vi "_CFX_Sole.vi"(0 "CFX cmd":T7, 1 "CFX State":T1, 5 "CFX-config":T3={"neme"="上板机", "CFX Handle"="Cleaner", "Request IP"="amqp://192.168.1.10:5672", "User"="admin", "password"="123456", "Broker IP"="192.168.1.20", "Broker Port"="5672", "Publish Path"="/exchange/Cleaner", "SubPubish Path"="/queue/Broadcast-Cleaner", "Broadcast \nPublish Path"="/exchange/CFX.Host", "Broadcast Sub\npublish Path"="/queue/Broadcast-CFX.Host", "Target \nHandle lD"="CFX.Host", "target IP"="amqp://127.0.0.1", "unit verification"=TRUE, "heartbeat"=FALSE, "timeout period"=5.0}, 7 "CfxData":T2={"Vendor"="YXD", "UniqueIdentifier"="UID5620001", "FriendlyName"="SBJ", "ModelNumber"="SBJ_0001", "SerialNumber"="563210", "NumberofLanes"="2", "CodeIn"="", "CodeOut"="", "Unitldentifer"="", "PositionNumber"="", "PositionName"="", "OldState"="", "NewState"="", "OldStateDuration"="", "Faultcode"="", "Operatorldentifer"="", "LoginName"="", "RecipeName"="", "Revision"="", "Activate formula"="", "Description"=""}, 11 "Error In":errorcluster caption="错误输入", 12 "send?":bool, 13 "request?":bool) -> (6 "MessageCFX_out":string, 8 "CFX_Message_In":T4, 14 "ok?":bool, 15 "Error Out":errorcluster caption="错误输出")   [LabVIEW 2025]
uses:
  CFX_dll/CFX.dll
  ctl/CFX-cmd.ctl
  ctl/CfxTopic-cmd.ctl
  ctl/CFX_data.ctl
  ctl/CFX-config.ctl
  SubVI/table/1 model/a log/_myType runlog cmd.ctl
panel:
  out "cmd State":T1=enum."Event"
  in  "Sole?":bool
  out "QueueName":string
  out "IsOpen":bool
  in  "CFX.Host?":bool
  in  "enable?":bool
  out "TraceMessage_EVE":refnum<k27>
  out "TraceMessage":string
  out "AooLog":refnum<k24>
  out "TestSubscribeChannel":bool
  out "TestPublishChannel":bool
  out "log":string
  out "error out":errorcluster
  out "objAMQP_MSG":refnum<k27>
  out "Connection":T5 {"ConnectionEstablished" items=["ConnectionEstablished", "ConnectionFailed", "ConnectionInterrupted", "ConnectionClosed"]}
  out "objAMQP_Request":refnum<k27>
  out "SubscribeChannel":refnum<k24>
  out "return":T6={"CFXHandle"="Cleaner", "RequestNetworkUri"="amqp://10.33.191.97:5672", "RequestTargetAddress"="/queue/Cleaner", "CFX_Message_In"={"Message_Name"="", "Message_Content"=""}, "CFX_Message_out"={"Message_Name"="", "Message_Content"=""}, "CFX_data"=refnum}
  out "FromListener":string
  in  "EndpointInformation":string
  in  "NewState":i32(ring)=1000 items=["PRD"=1000, "PRD_RegularWork"=1100, "PRD_WorkForThirdParties"=1200, "PRD_Rework"=1300, "PRD_Engineering"=1400, "SBY"=2000, "SBY_NoOperator"=2100, "SBY_NoProduct"=2200, "SBY_NoSupportTool"=2300, "SBY_AssociatedClusterModuleDown"=2400, "SBY_NoHost"=2500, "ENG"=3000, "ENG_ProcessExperiments"=3100, "ENG_EquipmentExperiments"=3200, "SDT"=4000, "SDT_UserMaintenanceDelay"=4100, "SDT_SuppliedMaintenanceDelay"=4200, "SDT_PreventiveMaintenance"=4300, "SDT_ChangeOfConsumables"=4400, "SDT_Setup"=4500, "SDT_ProductionTest"=4600, "SDT_FacilitiesRelated"=4700, "USD"=5000, "USD_UserMaintentanceDelay"=5100, "USD_SuppliedMaintenanceDelay"=5200, "USD_Repair"=5300, "USD_OutOfSpecInputMaterial"=5400, "USD_ChangeOfConsumables"=5500, "USD_FacilitiesRelated"=5600, "NST"=6000, "NST_UnworkedShifts"=6100, "NST_EquipmentInstallation"=6200, "NST_EquipmentModifications"=6300, "NST_OfflineTraining"=6400, "NST_ShutdownAndStartup"=6500]
  in  "Broker Url":string="amqp://admin:123456@10.33.191.54:5672"
  out "PublishChannel":refnum<k24>
  in  "rngNewState":i32(ring) items=["PRD"=1000, "PRD_RegularWork"=1100, "PRD_WorkForThirdParties"=1200, "PRD_Rework"=1300, "PRD_Engineering"=1400, "SBY"=2000, "SBY_NoOperator"=2100, "SBY_NoProduct"=2200, "SBY_NoSupportTool"=2300, "SBY_AssociatedClusterModuleDown"=2400, "SBY_NoHost"=2500, "ENG"=3000, "ENG_ProcessExperiments"=3100, "ENG_EquipmentExperiments"=3200, "SDT"=4000, "SDT_UserMaintenanceDelay"=4100, "SDT_SuppliedMaintenanceDelay"=4200, "SDT_PreventiveMaintenance"=4300, "SDT_ChangeOfConsumables"=4400, "SDT_Setup"=4500, "SDT_ProductionTest"=4600, "SDT_FacilitiesRelated"=4700, "USD"=5000, "USD_UserMaintentanceDelay"=5100, "USD_SuppliedMaintenanceDelay"=5200, "USD_Repair"=5300, "USD_OutOfSpecInputMaterial"=5400, "USD_ChangeOfConsumables"=5500, "USD_FacilitiesRelated"=5600, "NST"=6000, "NST_UnworkedShifts"=6100, "NST_EquipmentInstallation"=6200, "NST_EquipmentModifications"=6300, "NST_OfflineTraining"=6400, "NST_ShutdownAndStartup"=6500]
  # "此端点的唯一 CFX 句柄。"
  # "节点队列名"
  # "amqp://10.33.191.64:5672"
  # "Laser"
  # "amqp://localhost:5672"
  # "amqp://192.168.1.20:5672"
  # "Local Request Uri"
  # "amqp://10.33.191.64:5688"
  # "AMQP 源或目标的网络地址。可以包括 user 和 port 信息 标准 Uri 格式。（例如：amqps://user1:password1@myamqpbroker.company1.com、amqp://broker3.company1.com、 amqps://myamqpbroker.company1.com:8856 等）。"
  # "本地消息源\nRequest Source"
  # "代理层\nBroker"
  # "请求目标\nRequest Target"
  # "可配置项"
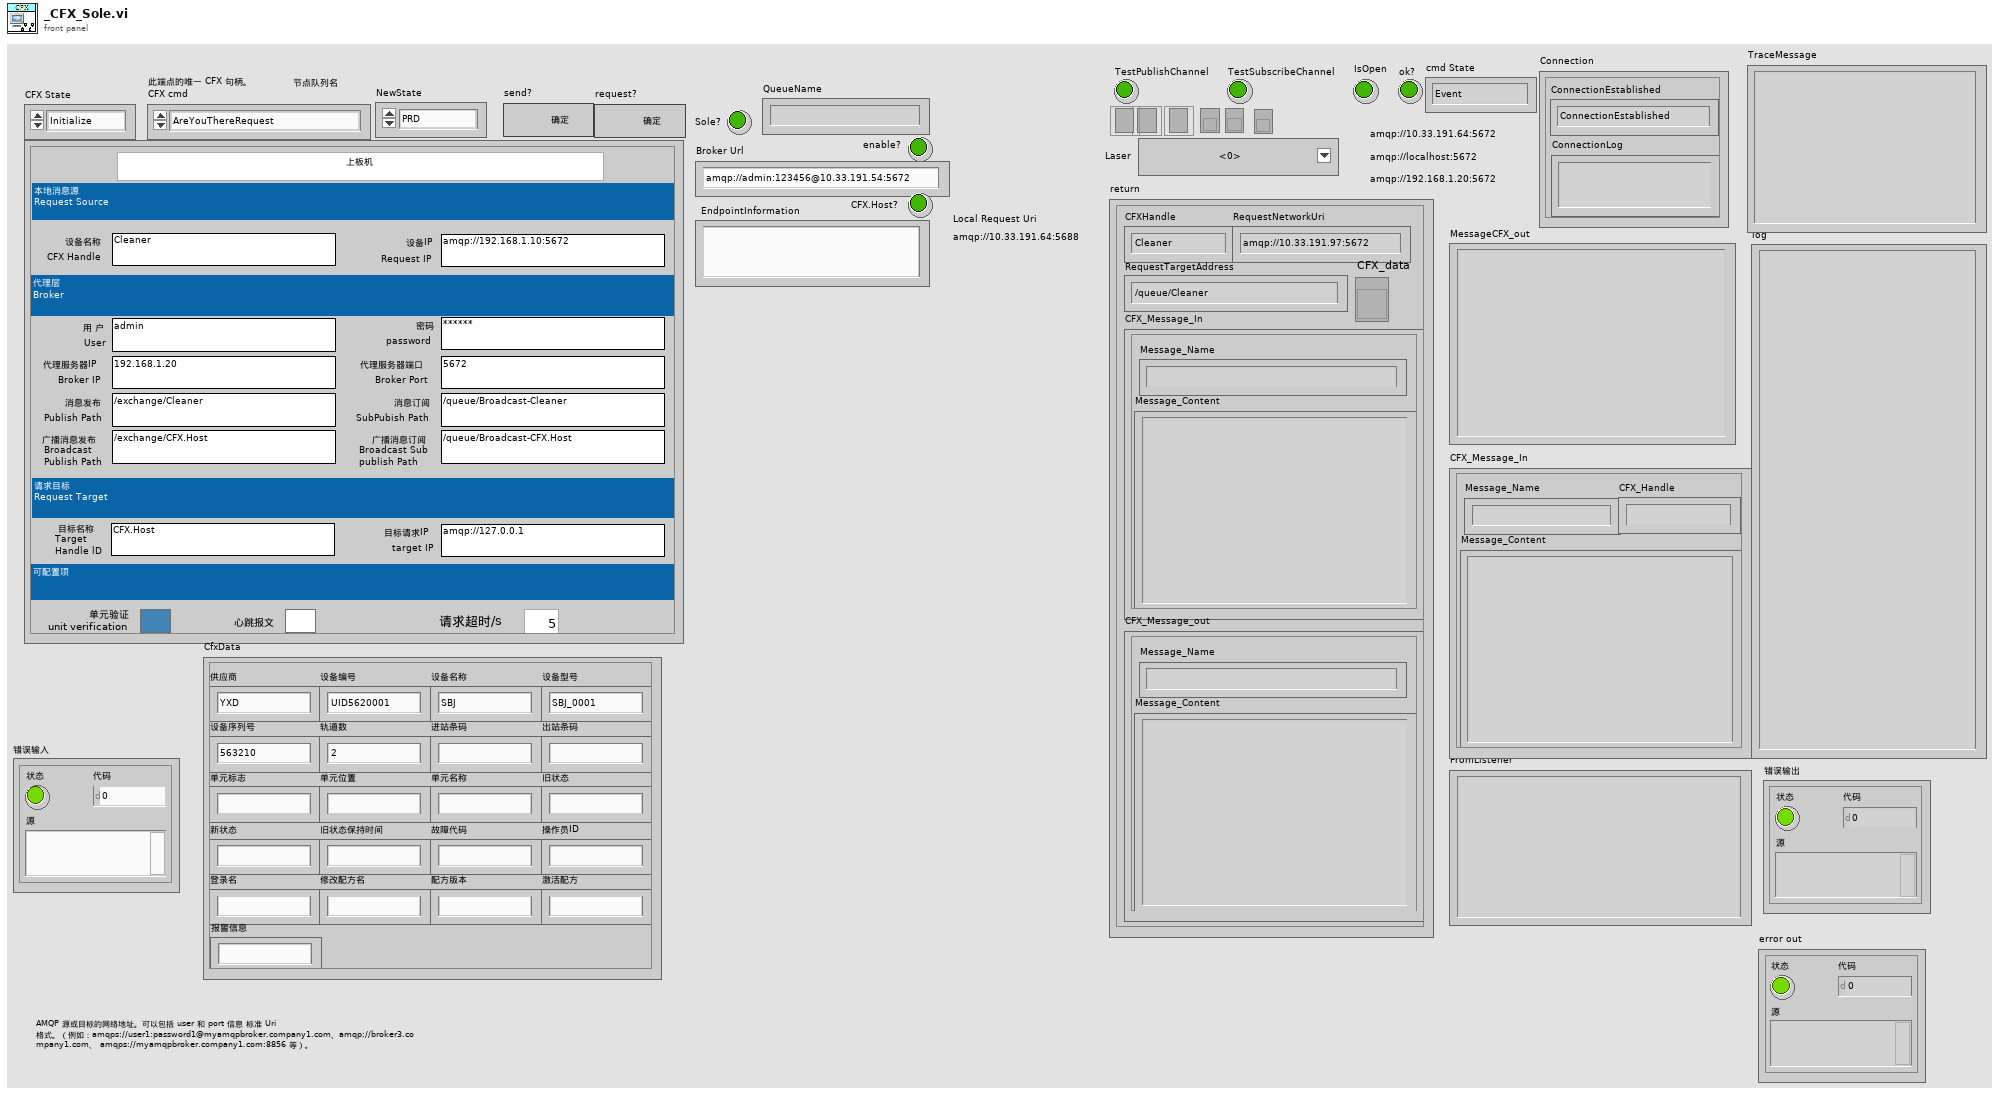
[diagram p1: front panel]
types:
  T1 = typedef "CFX-cmd.ctl" = enum16{"Initialize", "Event", "Connection test", "OpenConnection", "Idle", "Shutdown", "WorkComplete", "StationStateChanged", "MaterialsApplied", "CFX", "Hermes"}
  T2 = typedef "CFX_data.ctl" = cluster{"Vendor":string, "UniqueIdentifier":string, "FriendlyName":string, "ModelNumber":string, "SerialNumber":string, "NumberofLanes":string, "CodeIn":string, "CodeOut":string, "Unitldentifer":string, "PositionNumber":string, "PositionName":string, "OldState":string, "NewState":string, "OldStateDuration":string, "Faultcode":string, "Operatorldentifer":string, "LoginName":string, "RecipeName":string, "Revision":string, "Activate formula":string, "Description":string}
  T3 = typedef "CFX-config.ctl" = cluster{"neme":string, "CFX Handle":string, "Request IP":string, "User":string, "password":string, "Broker IP":string, "Broker Port":string, "Publish Path":string, "SubPubish Path":string, "Broadcast \nPublish Path":string, "Broadcast Sub\npublish Path":string, "Target \nHandle lD":string, "target IP":string, "unit verification":bool, "heartbeat":bool, "timeout period":dbl}
  T4 = cluster{"Message_Name":string, "CFX_Handle":string, "Message_Content":string}
  T5 = cluster{"ConnectionEstablished":i32, "ConnectionLog":string}
  T6 = cluster{"CFXHandle":string, "RequestNetworkUri":string, "RequestTargetAddress":string, "CFX_Message_In":cluster{"Message_Name":string, "Message_Content":string}, "CFX_Message_out":cluster{"Message_Name":string, "Message_Content":string}, "CFX_data":refnum<vi>}
  T7 = typedef "CfxTopic-cmd.ctl" = enum16{"AreYouThereRequest", "AreYouThereResponse", "EndpointConnected", "EndpointShuttingDown", "GetEndpointInformationRequest", "GetEndpointInformationResponse", "Heartbeat", "NotSupportedResponse", "WhoIsThereRequest", "WhoIsThereResponse", "UnitArrived", "UnitsDeparted", "StationStateChanged", "FaultOccurred", "FaultCleared", "OperatorActivated", "OperatorDeactivated", "RecipeModified", "RecipeActived", "ActivateRecipeRequest", "ActivateRecipeResponse"}
  T8 = typedef "_myType runlog cmd.ctl" = enum16{"init", "push (-1: error)", "push (0: user)", "push (1: logical)", "push (2: driver)", "push (3: lib-core)", "push (4: reserved)", "pop", "more?"}
  T9 = typedef "LVStringsAndValuesArrayTypeDef_I32.ctl" = cluster{"String":string, "Value":i32}[]
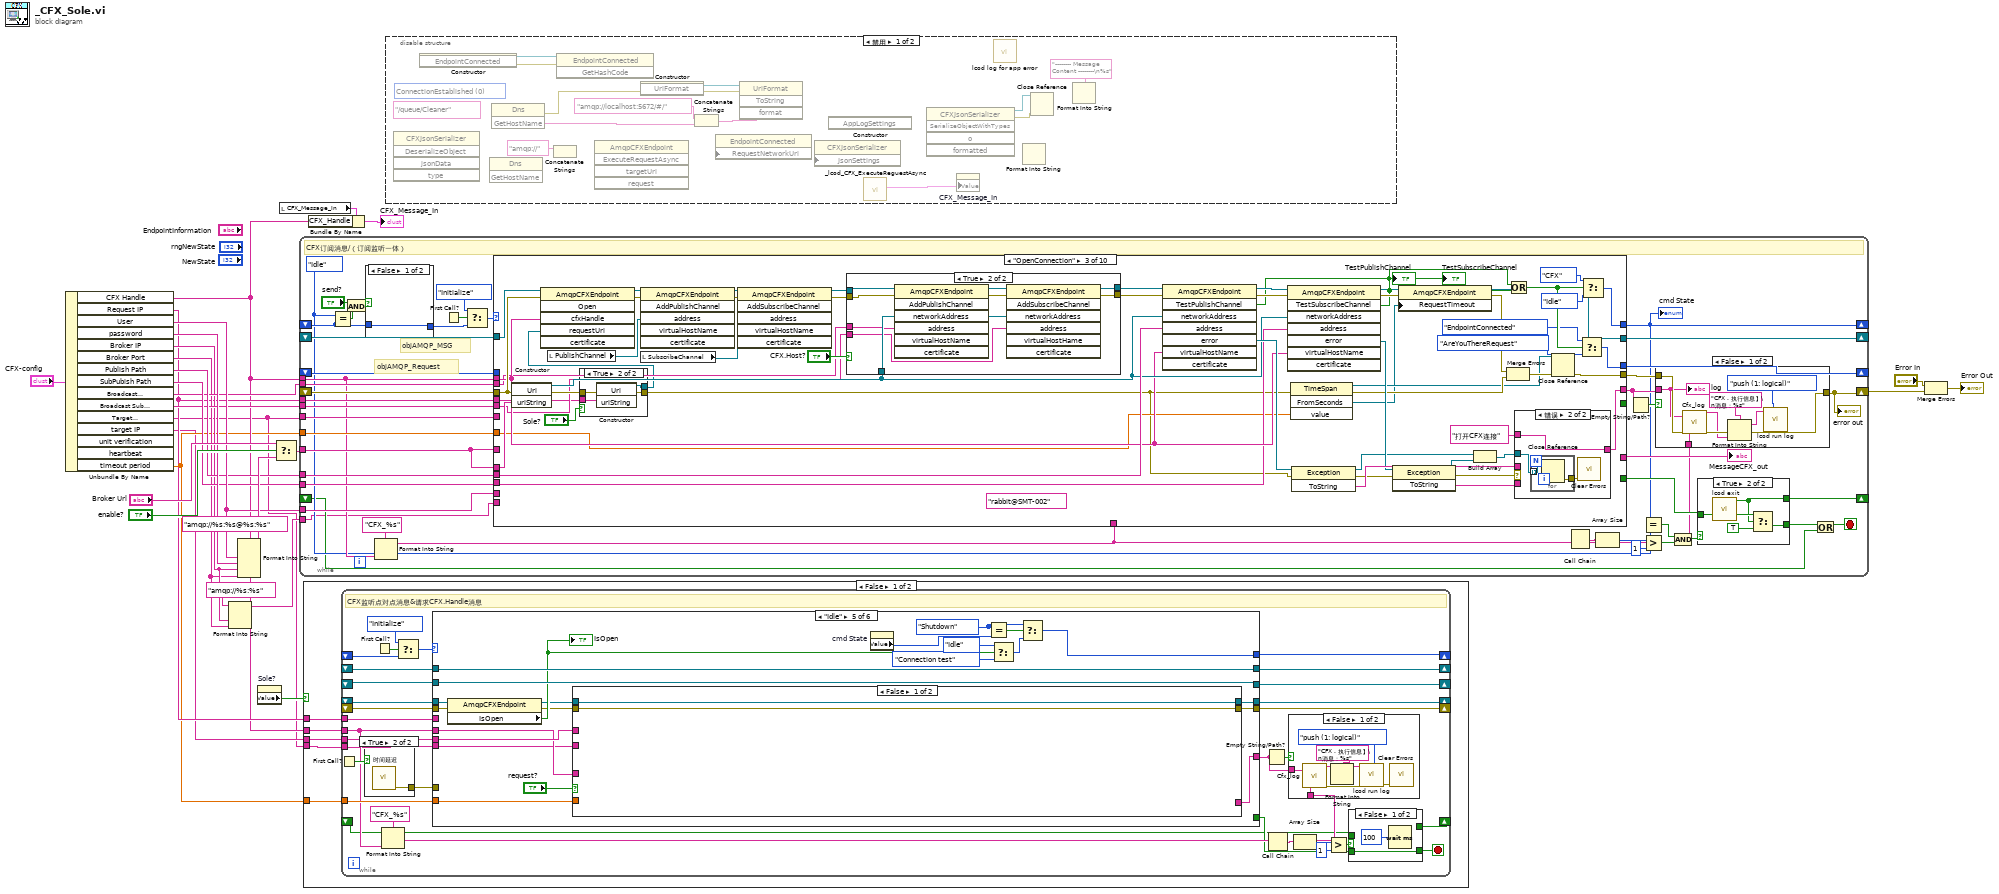
[diagram p0: block diagram]
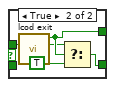
[diagram p2: hidden frame]
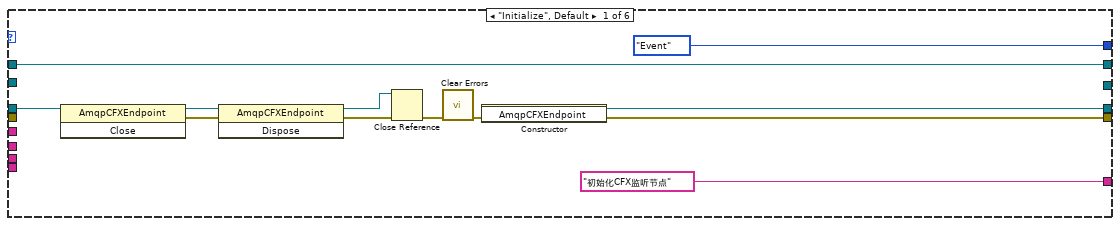
[diagram p5: hidden frame]
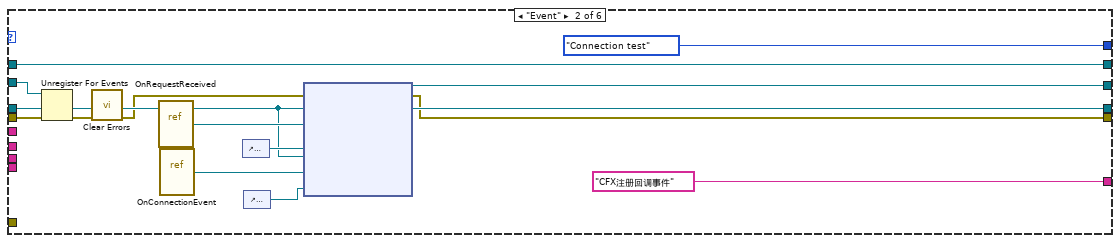
[diagram p6: hidden frame]
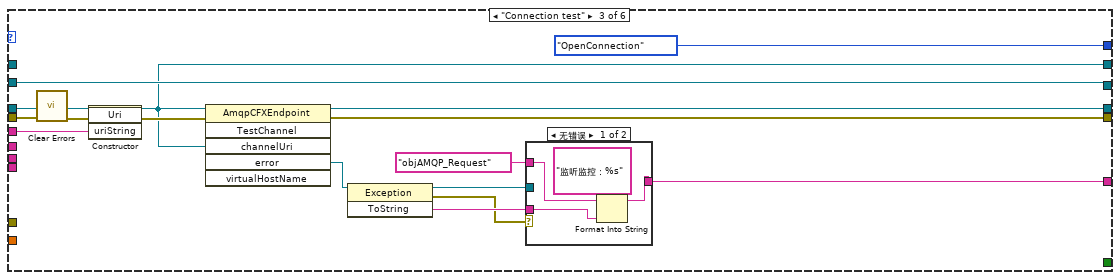
[diagram p7: hidden frame]
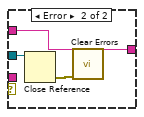
[diagram p8: hidden frame]
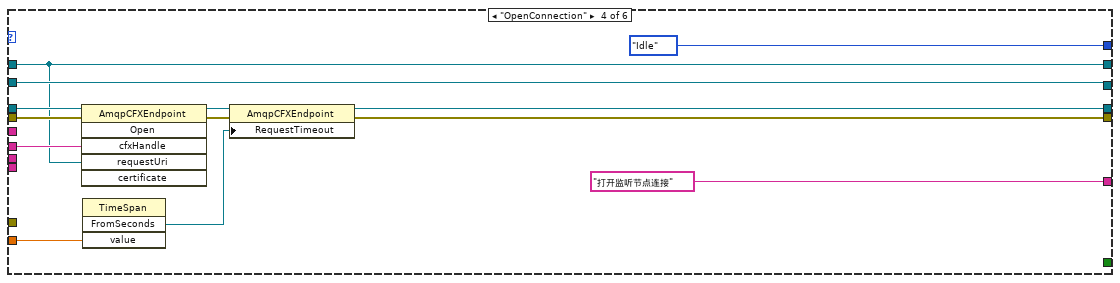
[diagram p9: hidden frame]
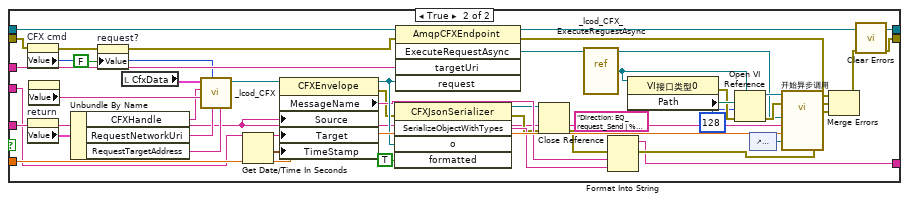
[diagram p10: hidden frame]
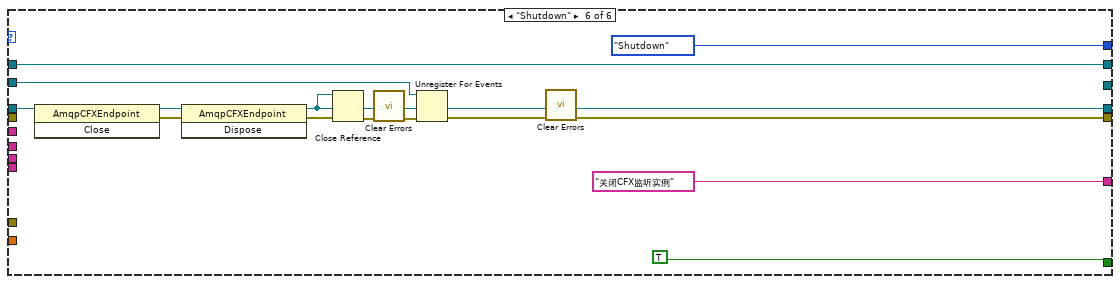
[diagram p11: hidden frame]
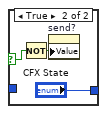
[diagram p14: hidden frame]
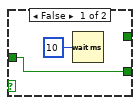
[diagram p15: hidden frame]
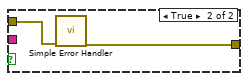
[diagram p16: hidden frame]
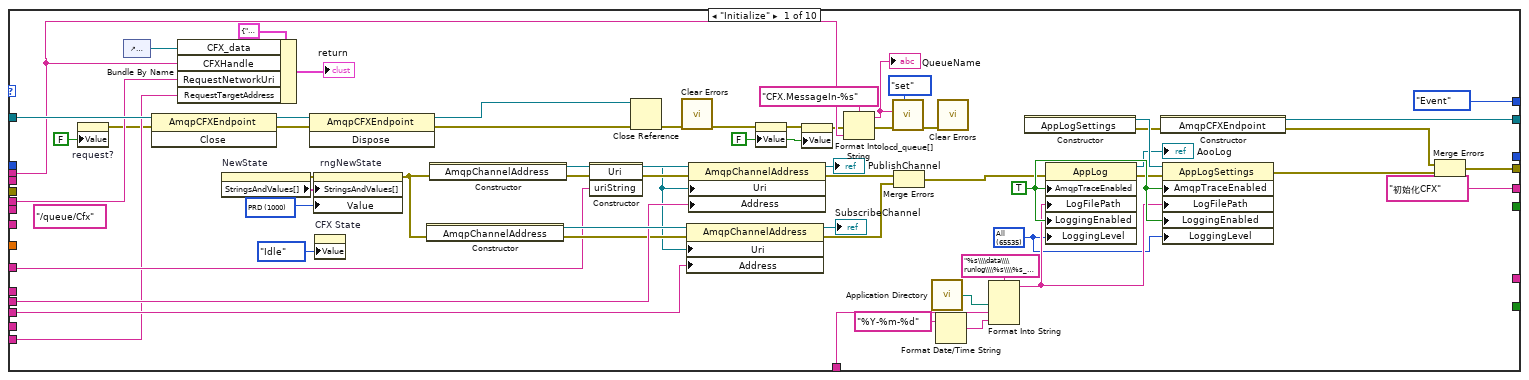
[diagram p17: hidden frame]
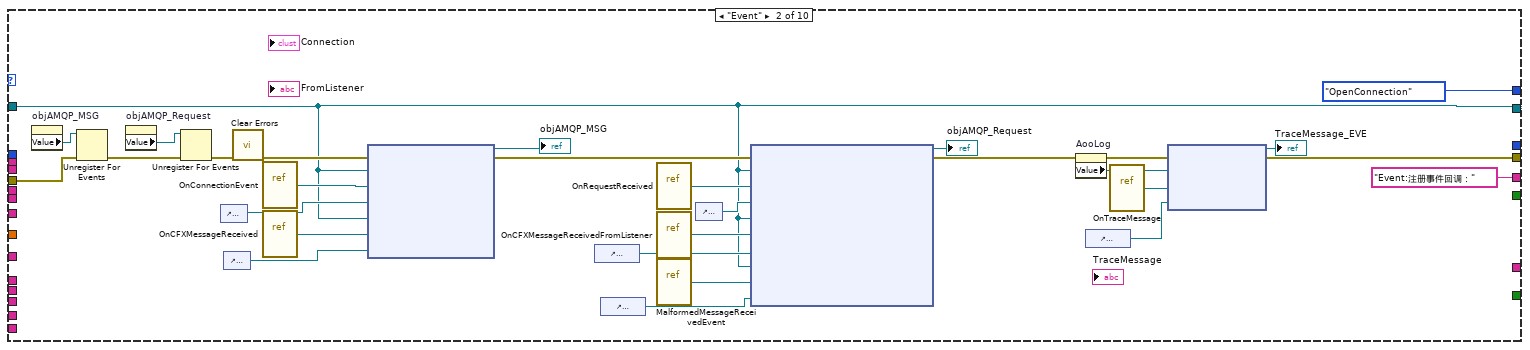
[diagram p18: hidden frame]
diagram:
  n1 = Unbundle By Name("CFX-config") -> ("CFX Handle"=w5:string, "Request IP"=w6:string, "User"=w20:string, "password"=w19:string, "Broker IP"=w10:string, "Broker Port"=w9:string, "Publish Path"=w18:string, "SubPubish Path"=w17:string, "Broadcast \nPublish Path"=w16:string, "Broadcast Sub\npublish Path"=w15:string, "Target \nHandle lD"=w1:string, "target IP"=w2:string, "timeout period"=w4:dbl)  [unwired: 2 out]
  n2 = Format Into String(format string="amqp://%s:%s" ("格式字符串"), w10, w9) -> (resulting string=w8:string)  [unwired: 2 in, 1 out]
  n3 = Format Into String(format string="amqp://%s:%s@%s:%s" ("格式字符串"), w20, w19, w10, w9) -> (resulting string=w22:string)  [unwired: 2 in, 1 out]
  n4 = property on="Sole?" class="Bool (严格)"() -> ("Value"=w3:bool)  [unwired: 2 in, 2 out]
  n5 = Select(t="Broker Url", s="enable?", f=w22) -> (s? t:f=w14:string)
  n6 = local read "CFX_Message_In"() -> (w13:T4)
  n7 = while {
    shift-right: [w47] -> _
    shift-left: _ -> [w36]
    shift-right: [w70] -> _
    shift-left: _ -> [w71]
    shift-right: [w64] -> w7
    shift-left: _ -> [w58]
    shift-right: [w63] -> _
    shift-left: _ -> [w65]
    tunnel: w14 -> [w59]
    tunnel: w17 -> [w62]
    tunnel: w18 -> [w61]
    tunnel: w5 -> [w41]
    tunnel: w20 -> [w60]
    tunnel: w6 -> [w57]
    tunnel: w16 -> [w56]
    tunnel: w15 -> [w55]
    tunnel: w1 -> [w54]
    tunnel: w4 -> [w53]
    shift-right: [w37] -> _
    shift-left: _ -> [w31]
    tunnel: w8 -> [w28]
    stop <- w32 stop-if-true
    w35 = CFX-cmd."Idle" ("CFX State")
    # "objAMQP_Request"
    # "objAMQP_MSG"
    # "CFX订阅消息/（订阅监听一体）"
    n8 = Equal?(x=w35, y=w36) -> (x = y?=w33:bool)
    n9 = And(x="send?", y=w33) -> (x .and. y?=w34:bool)
    n10 = case shown="False" w34 {
      selector: w34 -> [_ w74]
      tunnel: w36 -> [w72 _]
      tunnel: [w72 "CFX State"] -> w40
      frame False {
      }
      frame True {
        n11 = Not(x=w74) -> (.not. x?=w73:bool)
        n12 = property on="send?" class="Bool (严格)"("Value"=w73) -> ()  [unwired: 2 in, 2 out]
      }
    }
    n13 = Format Into String(format string="CFX_%s" ("log_path"), w41) -> (resulting string=w39:string)  [unwired: 2 in, 1 out]
    n14 = First Call?() -> (First Call?: T/F=w29:bool)
    n15 = Select(t=CFX-cmd."Initialize" ("CFX State"), s=w29, f=w40) -> (s? t:f=w43:T1)
    n16 = case shown="\"OpenConnection\"" w43 {
      selector: w43 -> [_ _ _ w294 _ _ _ _ _ _]
      tunnel: [_ _ _ _ w340 _ _ _ _ _] -> w49
      tunnel: w71 -> [w132 w153 w237 w283 w346 w390 w418 w443 w483 w501]
      tunnel: [w138 w153 w194 w269 w342 w389 w416 w442 w482 w500] -> w70
      tunnel: [w133 w172 w208 errorcluster {"status"=FALSE, "code"=0, "source"=""} ("error out") w341 w386 w413 w441 w493 w499] -> w69
      tunnel: [_ _ _ w293 _ w381 w405 w428 w477 w498] -> w68
      tunnel: [_ _ _ TRUE _ _ _ _ _ _] -> _
      tunnel: ["初始化CFX" ("格式字符串") "Event:注册事件回调：" ("SerializeObjectWithTypes") w230 "" ("SerializeObjectWithTypes") w345 w378 w405 w427 w487 w498] -> w67
      tunnel: [CFX-cmd."Event" ("CFX State") CFX-cmd."OpenConnection" ("CFX State") w201 w278 w344 CFX-cmd."Idle" ("CFX State") CFX-cmd."Idle" ("CFX State") CFX-cmd."Idle" ("CFX State") w463 CFX-cmd."Idle" ("CFX State")] -> w47
      tunnel: w58 -> [_ w167 w211 w266 w343 w376 w403 w425 w484 w496]
      tunnel: w65 -> [_ _ _ _ w339 _ _ _ w467 _]
      tunnel: [_ _ w197 w288 w336 _ _ _ w462 _] -> w63
      tunnel: w59 -> [w105 _ _ _ _ _ _ _ _ _]
      tunnel: w62 -> [w123 _ w190 _ _ _ _ _ _ _]
      tunnel: w61 -> [w122 _ w220 w285 _ _ _ _ _ _]
      tunnel: w41 -> [w108 _ w204 _ _ _ _ _ w460 _]
      tunnel: w60 -> [_ _ _ w284 _ _ _ _ _ _]
      tunnel: w59 -> [_ _ w219 _ _ _ _ _ _ _]
      tunnel: w57 -> [w109 _ w188 _ _ _ _ _ _ _]
      tunnel: w56 -> [_ _ w192 _ _ _ _ _ _ _]
      tunnel: w55 -> [_ _ w191 _ _ _ _ _ _ _]
      tunnel: w54 -> [_ _ _ _ _ _ _ _ w459 _]
      tunnel: w53 -> [_ _ w189 _ _ _ _ _ _ _]
      tunnel: w39 -> [w107 _ _ _ _ _ _ _ _ _]
      tunnel: w28 -> [w98 _ _ _ _ _ _ _ _ _]
      frame "Initialize" {
        (unwired) "/queue/Cfx" ("RequestTargetAddress")
        w127 = FALSE ("TestPublishChannel")
        w135 = 65535 items=["Debug"=1, "Info"=2, "Warn"=4, "Error"=8, "All"=65535] ("LoggingLevel")
        w137 = TRUE ("LoggingEnabled")
        w149 = 1000 items=["PRD"=1000, "PRD_RegularWork"=1100, "PRD_WorkForThirdParties"=1200, "PRD_Rework"=1300, "PRD_Engineering"=1400, "SBY"=2000, "SBY_NoOperator"=2100, "SBY_NoProduct"=2200, "SBY_NoSupportTool"=2300, "SBY_AssociatedClusterModuleDown"=2400, "SBY_NoHost"=2500, "ENG"=3000, "ENG_ProcessExperiments"=3100, "ENG_EquipmentExperiments"=3200, "SDT"=4000, "SDT_UserMaintenanceDelay"=4100, "SDT_SuppliedMaintenanceDelay"=4200, "SDT_PreventiveMaintenance"=4300, "SDT_ChangeOfConsumables"=4400, "SDT_Setup"=4500, "SDT_ProductionTest"=4600, "SDT_FacilitiesRelated"=4700, "USD"=5000, "USD_UserMaintentanceDelay"=5100, "USD_SuppliedMaintenanceDelay"=5200, "USD_Repair"=5300, "USD_OutOfSpecInputMaterial"=5400, "USD_ChangeOfConsumables"=5500, "USD_FacilitiesRelated"=5600, "NST"=6000, "NST_UnworkedShifts"=6100, "NST_EquipmentInstallation"=6200, "NST_EquipmentModifications"=6300, "NST_OfflineTraining"=6400, "NST_ShutdownAndStartup"=6500] ("NewState")
        n17 = property on="request?" class="Bool (严格)"("Value"=FALSE ("request?")) -> (error out=w93:errorcluster)  [unwired: 2 in, 1 out]
        n18 = control-ref of="CfxData"() -> (w95:refnum<vi>)
        n19 = invoke class="AmqpCFXEndpoint" method="Close"(reference=w132, error in=w93) -> (reference out=w130:refnum<k24>, error out=w99:errorcluster)  [unwired: 1 in, 1 out]
        n20 = Bundle By Name(cluster=T6 {"CFXHandle"="Cleaner", "RequestNetworkUri"="amqp://192.168.1.10:5672", "RequestTargetAddress"="/queue/Cleaner", "CFX_Message_In"={"Message_Name"="", "Message_Content"=""}, "CFX_Message_out"={"Message_Name"="", "Message_Content"=""}, "CFX_data"=refnum} ("return"), "CFX_data"=w95, "CFXHandle"=w108, "RequestNetworkUri"=w109, "RequestTargetAddress"=w98) -> (→"return":T6)
        n21 = property on="NewState" class="Ring (严格)"() -> (error out=w148:errorcluster, "StringsAndValues[]"=w152:T9)  [unwired: 2 in, 1 out]
        n22 = invoke on="调用节点" class="AmqpCFXEndpoint" method="Dispose"(reference=w130, error in=w99) -> (reference out=w101:refnum<k24>, error out=w100:errorcluster)  [unwired: 1 in, 1 out]
        n23 = property on="rngNewState" class="Ring (严格)"(error in=w148, "StringsAndValues[]"=w152, "Value"=w149) -> (error out=w129:errorcluster)  [unwired: 1 in, 1 out]
        n24 = property on="CFX State" class="Enum (严格)"("Value"=CFX-cmd."Idle" ("CFX State")) -> ()  [unwired: 2 in, 2 out]
        n25 = constructor class="AmqpChannelAddress"(error in=w129) -> (reference out=w142:refnum<k24>, error out=w121:errorcluster)  [unwired: 2 in, 1 out]
        n26 = constructor class="AmqpChannelAddress"(error in=w129) -> (reference out=w147:refnum<k24>, error out=w151:errorcluster)  [unwired: 2 in, 1 out]
        n27 = constructor class="Uri"(error in=w151, "uriString"=w105) -> (reference out=w120:refnum<k24>, error out=w150:errorcluster)  [unwired: 2 in, 2 out]
        n28 = Close Reference(reference=w101, error in (no error)=w100) -> (error out=w131:errorcluster)
        n29 = call <vilib>:"Clear Errors.vi"("error in (no error)"=w131) -> ("error out"=w119:errorcluster)  [unwired: 5 in, 1 out]
        n30 = property class="AmqpChannelAddress"(reference=w142, error in=w121, "Uri"=w120, "Address"=w123) -> (reference out=→"SubscribeChannel":refnum<k24>, error out=w140:errorcluster)
        n31 = property class="AmqpChannelAddress"(reference=w147, error in=w150, "Uri"=w120, "Address"=w122) -> (reference out=→"PublishChannel":refnum<k24>, error out=w141:errorcluster)
        n32 = property on="TestPublishChannel" class="Bool (严格)"(error in=w119, "Value"=w127) -> (error out=w128:errorcluster)  [unwired: 1 in, 1 out]
        n33 = property on="TestSubscribeChannel" class="Bool (严格)"(error in=w128, "Value"=w127) -> (error out=w104:errorcluster)  [unwired: 1 in, 1 out]
        n34 = Format Into String(format string="CFX.MessageIn-%s" ("格式字符串"), error in=w104, w108) -> (resulting string=w113:string, error out=w110:errorcluster)  [unwired: 1 in]
        "QueueName" <- w113
        n35 = call "locd_queue[].vi"("cmd"=enum16{"init", "get", "set", "end"}."set", "error in"=w110, "queue_name"=w113) -> ("error out"=w111:errorcluster)  [unwired: 4 in, 4 out]
        n36 = Merge Errors(w141, w140) -> (w112:errorcluster)
        n37 = call <vilib>:"Application Directory.vi"() -> ("Application Directory"=w146:path)
        n38 = Format Date/Time String(time format string (%c)="%Y-%m-%d" ("格式字符串")) -> (date/time string=w106:string)  [unwired: 2 in]
        n39 = call <vilib>:"Clear Errors.vi"("error in (no error)"=w111) -> ()  [unwired: 5 in, 2 out]
        n40 = Format Into String(format string="%s\\\\data\\\\runlog\\\\%s\\\\%s_cfxDebig.txt" ("格式字符串"), w146, w107, w106) -> (resulting string=w136:string)  [unwired: 2 in, 1 out]
        n41 = constructor class="AppLogSettings"() -> (reference out=w134:refnum<k24>, error out=w126:errorcluster)  [unwired: 3 in, 1 out]
        n42 = property class="AppLog"(error in=w112, "AmqpTraceEnabled"=w137, "LogFilePath"=w136, "LoggingEnabled"=w137, "LoggingLevel"=w135) -> (reference out=→"AooLog":refnum<k24>, error out=w124:errorcluster)  [unwired: 1 in]
        n43 = constructor class="AmqpCFXEndpoint"(error in=w126) -> (reference out=w138:refnum<k24>, error out=w102:errorcluster)  [unwired: 2 in, 1 out]
        n44 = property class="AppLogSettings"(reference=w134, error in=w124, "AmqpTraceEnabled"=w137, "LogFilePath"=w136, "LoggingEnabled"=w137, "LoggingLevel"=w135) -> (error out=w116:errorcluster)  [unwired: 1 out]
        n45 = Merge Errors(w102, w116) -> (w133:errorcluster)
      }
      frame "Event" {
        n46 = property on="objAMQP_MSG" class="Ref (严格)"() -> ("Value"=w156:refnum<k27>)  [unwired: 2 in, 2 out]
        n47 = Unregister For Events(event registration refnum=w156, error in=w167) -> (error out=w157:errorcluster)
        n48 = property on="objAMQP_Request" class="Ref (严格)"() -> ("Value"=w154:refnum<k27>)  [unwired: 2 in, 2 out]
        n49 = Unregister For Events(event registration refnum=w154, error in=w157) -> (error out=w155:errorcluster)
        n50 = control-ref of="Connection"() -> (w179:refnum<vi>)
        n51 = control-ref of="CFX_Message_In"() -> (w164:refnum<vi>)
        n52 = call <vilib>:"Clear Errors.vi"("error in (no error)"=w155) -> ("error out"=w158:errorcluster)  [unwired: 5 in, 1 out]
        n53 = vi-ref "OnConnectionEvent.vi"() -> ("vi reference"=w180:refnum<vi>)
        n54 = vi-ref "OnCFXMessageReceived.vi"() -> ("vi reference"=w165:refnum<vi>)
        n55 = node(w158, w153, w180, w179, w153, w165, w164) -> (→"objAMQP_MSG":refnum<k27>, w163:errorcluster)  [unwired: 1 in]
        n56 = control-ref of="FromListener"() -> (w161:refnum<vi>)
        n57 = control-ref of="FromListener"() -> (w159:refnum<vi>)
        n58 = vi-ref "OnRequestReceived.vi"() -> ("vi reference"=w178:refnum<vi>)
        n59 = vi-ref "OnCFXMessageReceivedFromListener.vi"() -> ("vi reference"=w162:refnum<vi>)
        n60 = vi-ref "MalformedMessageReceivedEvent.vi"() -> ("vi reference"=w160:refnum<vi>)
        n61 = control-ref of="return"() -> (w169:refnum<vi>)
        n62 = node(w163, w153, w178, w169, w153, w162, w161, w153, w160, w159) -> (→"objAMQP_Request":refnum<k27>, w166:errorcluster)  [unwired: 1 in]
        n63 = property on="AooLog" class="Ref (严格)"(error in=w166) -> (error out=w168:errorcluster, "Value"=w174:refnum<k24>)  [unwired: 1 in, 1 out]
        n64 = control-ref of="TraceMessage"() -> (w170:refnum<vi>)
        n65 = vi-ref "OnTraceMessage.vi"() -> ("vi reference"=w173:refnum<vi>)
        n66 = node(w168, w174, w173, w170) -> (→"TraceMessage_EVE":refnum<k27>, w172:errorcluster)  [unwired: 1 in]
      }
      frame "OpenConnection" {
        (unwired) "rabbit@SMT-002" ("sourceAddress")
        n67 = constructor class="Uri"(error in=w211, "uriString"=w219) -> (reference out=w218:refnum<k24>, error out=w216:errorcluster)  [unwired: 2 in, 2 out]
        n68 = local read "PublishChannel"() -> (w232:refnum<k24>)
        n69 = case shown="True" "Sole?" {
          tunnel: w216 -> [w238 w242]
          tunnel: w188 -> [_ w241]
          tunnel: [_ w240] -> w184
          tunnel: [w238 w239] -> w183
          frame False {
          }
          frame True {
            n70 = constructor class="Uri"(error in=w242, "uriString"=w241) -> (reference out=w240:refnum<k24>, error out=w239:errorcluster)  [unwired: 2 in, 2 out]
          }
        }
        n71 = invoke class="AmqpCFXEndpoint" method="Open"(reference=w237, error in=w211, "cfxHandle"=w204, "requestUri"=w184) -> (reference out=w215:refnum<k24>, error out=w214:errorcluster)  [unwired: 2 in, 4 out]
        n72 = local read "SubscribeChannel"() -> (w233:refnum<k24>)
        n73 = invoke class="AmqpCFXEndpoint" method="AddPublishChannel"(reference=w215, error in=w214, "address"=w232) -> (reference out=w236:refnum<k24>, error out=w235:errorcluster)  [unwired: 3 in, 4 out]
        n74 = invoke class="AmqpCFXEndpoint" method="AddSubscribeChannel"(reference=w236, error in=w235, "address"=w233) -> (reference out=w212:refnum<k24>, error out=w205:errorcluster)  [unwired: 3 in, 4 out]
        n75 = case shown="True" "CFX.Host?" {
          tunnel: w218 -> [_ w253]
          tunnel: [w243 w252] -> w217
          tunnel: [w244 w251] -> w213
          tunnel: w212 -> [w244 w250]
          tunnel: w205 -> [w243 w247]
          tunnel: w192 -> [_ w246]
          tunnel: w191 -> [_ w245]
          frame False {
          }
          frame True {
            n76 = invoke class="AmqpCFXEndpoint" method="AddPublishChannel"(reference=w250, error in=w247, "networkAddress"=w253, "address"=w246) -> (reference out=w248:refnum<k24>, error out=w249:errorcluster)  [unwired: 3 in, 5 out]
            n77 = invoke class="AmqpCFXEndpoint" method="AddSubscribeChannel"(reference=w248, error in=w249, "networkAddress"=w253, "address"=w245) -> (reference out=w251:refnum<k24>, error out=w252:errorcluster)  [unwired: 3 in, 5 out]
          }
        }
        n78 = invoke on="调用节点" class="AmqpCFXEndpoint" method="TestPublishChannel"(reference=w213, error in=w217, "networkAddress"=w218, "address"=w220, "virtualHostName"=w204) -> (reference out=w231:refnum<k24>, error out=w222:errorcluster, "TestPublishChannel"=w203:bool, "error"=w228:refnum<k24>)  [unwired: 3 in, 4 out]
        "TestPublishChannel" <- w203
        n79 = invoke on="调用节点" class="AmqpCFXEndpoint" method="TestSubscribeChannel"(reference=w231, error in=w222, "networkAddress"=w218, "address"=w190, "virtualHostName"=w204) -> (reference out=w229:refnum<k24>, error out=w210:errorcluster, "TestSubscribeChannel"=w202:bool, "error"=w225:refnum<k24>)  [unwired: 3 in, 4 out]
        "TestSubscribeChannel" <- w202
        n80 = invoke class="TimeSpan" method="FromSeconds"(error in=w183, "value"=w189) -> (reference out=w207:refnum<k24>, error out=w209:errorcluster, "FromSeconds"=w193:refnum<k24>)  [unwired: 2 in, 1 out]
        n81 = invoke class="Exception" method="ToString"(reference=w228, error in=w183) -> (reference out=w187:refnum<k24>, error out=w226:errorcluster, "ToString"=w227:string)  [unwired: 1 in]
        n82 = invoke class="Exception" method="ToString"(reference=w225, error in=w226) -> (reference out=w186:refnum<k24>, error out=w223:errorcluster, "ToString"=w224:string)  [unwired: 1 in]
        n83 = property on="属性节点" class="AmqpCFXEndpoint"(reference=w229, "RequestTimeout"=w193) -> (reference out=w194:refnum<k24>)  [unwired: 1 in, 1 out]
        n84 = Build Array(w187, w186) -> (w185:refnum<k24>[])
        n85 = Merge Errors(w210, w209) -> (w221:errorcluster)
        n86 = Or(x=w203, y=w202) -> (x .or. y?=w198:bool)
        n87 = case shown="错误" w223 {
          tunnel: "打开CFX连接" ("格式字符串") -> [w258 w261]
          tunnel: [w257 w261] -> w230
          tunnel: w227 -> [w255 _]
          tunnel: w224 -> [w254 _]
          tunnel: w185 -> [_ w260]
          frame No Error {
            n88 = Format Into String(format string="发布：%s\n订阅：%s" ("格式字符串"), initial string=w258, w255, w254) -> (resulting string=w257:string)  [unwired: 1 in, 1 out]
          }
          frame Error {
            n89 = for {
              tunnel: w260 -> [w263] mode=indexing
              tunnel: [w262] -> w259
              n90 = Close Reference(reference=w263) -> (error out=w262:errorcluster)  [unwired: 1 in]
            }
            n91 = call <vilib>:"Clear Errors.vi"("error in (no error)"=w259) -> ()  [unwired: 5 in, 2 out]
          }
        }
        n92 = Close Reference(reference=w207, error in (no error)=w221) -> (error out=w208:errorcluster)
        n93 = Select(t=CfxTopic-cmd."EndpointConnected" ("CFX cmd"), s=w198, f=CfxTopic-cmd."AreYouThereRequest") -> (s? t:f=w197:T7)
        n94 = Select(t=CFX-cmd."CFX" ("CFX State"), s=w198, f=CFX-cmd."Idle" ("CFX State")) -> (s? t:f=w201:T1)
      }
      frame "Idle", Default {
        n95 = property on="属性节点" class="AmqpCFXEndpoint"(reference=w283, error in=w266) -> (reference out=w269:refnum<k24>, error out=w265:errorcluster, "IsOpen"=w282:bool)
        n96 = local read "IsOpen"() -> (w267:bool)
        n97 = And(x=w282, y=w267) -> (x .and. y?=→"ok?":bool)
        n98 = property on="CFX_Message_In" class="Clust (严格)"(error in=w265) -> (error out=w281:errorcluster, "Value"=w273:T4)  [unwired: 1 in, 1 out]
        n99 = feedback-in #1(w273) -> ()
        n100 = feedback #1() -> (w286:T4)  [unwired: 1 in]
        n101 = Not Equal?(x=w273, y=T4 {"Message_Name"="", "CFX_Handle"="", "Message_Content"=""} ("CFX_Message_In")) -> (x != y?=w271:bool)
        n102 = Not Equal?(x=w273, y=w286) -> (x != y?=w277:bool)
        n103 = And(x=w277, y=w271) -> (x .and. y?=w272:bool)
        n104 = property on="QueueName" class="Str"() -> ("Value"=w274:string)  [unwired: 2 in, 2 out]
        n105 = Build Array(w272) -> (w275:bool[])
        n106 = Boolean Array To Number(Boolean array=w275) -> (number=w276:u32)
        n107 = case shown="1" w276 {
          tunnel: [_ w301 _] -> w288
          tunnel: [CFX-cmd."Idle" ("CFX State") w300 CFX-cmd."Idle" ("CFX State")] -> w287
          tunnel: w285 -> [_ _ _]
          tunnel: w284 -> [_ _ _]
          tunnel: w273 -> [_ w298 _]
          tunnel: w281 -> [_ w296 w326]
          tunnel: w274 -> [_ w297 w324]
          frame 0, Default {
          }
          frame 1 {
            n108 = disable-structure shown="禁用" {
              disable-tunnel: w298 -> [w314 _]
              disable-tunnel: w297 -> [w304 _]
              disable-tunnel: w296 -> [w303 _]
              frame Disabled {
                n109 = Unbundle By Name(w314) -> ("Message_Name"=w313:string, "Message_Content"=w312:string)
                n110 = call "locd_queue[].vi"("cmd"=enum16{"init", "get", "set", "end"}."get", "error in"=w303, "queue_name"=w304) -> ("error out"=w315:errorcluster, "queue_out"=w317:refnum<queue>)  [unwired: 4 in, 3 out]
                n111 = To Variant(anything=w314) -> (Variant=w316:variant)
                n112 = call "Cfx_log.vi"("R/W"=enum16{"Send", "Receive"}."Receive", "Message_Name"=w313, "Message_Content"=w312) -> ("Log_out"=w306:string)  [unwired: 15 in, 1 out]
                n113 = Enqueue Element(queue=w317, element=w316, timeout in ms (-1)=100 ("超时毫秒(-1)"), error in (no error)=w315) -> (error out=w302:errorcluster)  [unwired: 2 out]
                n114 = Format Into String(format string="CFX . 执行信息】\n消息：%s", w306) -> (resulting string=w309:string, error out=w310:errorcluster)  [unwired: 2 in]
                n115 = call <vilib>:"Clear Errors.vi"("error in (no error)"=w302) -> ()  [unwired: 5 in, 2 out]
                n116 = call "lcod run log.vi"("cmd"=_myType_runlog_cmd."push (1: logical)", "Error In"=w310, "str in"=w309) -> ()  [unwired: 6 in, 3 out]
              }
              frame Enabled {
              }
            }
            n117 = property on="Message_Name" class="Str"() -> ("Value"=w299:string)  [unwired: 2 in, 2 out]
            n118 = case shown="\"\", 默认" w299 {
              tunnel: [_ CfxTopic-cmd."AreYouThereRequest" ("CFX cmd") CfxTopic-cmd."WhoIsThereResponse" ("CFX cmd")] -> w301
              tunnel: [w319 CFX-cmd."CFX" ("CFX State") CFX-cmd."CFX" ("CFX State")] -> w300
              frame "", Default {
                n119 = local read "CFX State"() -> (w319:T1)
              }
              frame "CFX.EndpointConnected" {
              }
              frame "CFX.WhoIsThereRequest" {
              }
            }
          }
          frame 2 {
            n120 = disable-structure shown="禁用" {
              disable-tunnel: w326 -> [w332 _]
              disable-tunnel: w324 -> [w327 _]
              frame Disabled {
                n121 = property on="return" class="Clust (严格)"(error in=w332) -> (error out=w334:errorcluster, "Value"=w333:T6)  [unwired: 1 in, 1 out]
                n122 = call "locd_queue[].vi"("cmd"=enum16{"init", "get", "set", "end"}."get", "queue_name"=w327) -> ("queue_out"=w331:refnum<queue>)  [unwired: 5 in, 4 out]
                n123 = To Variant() -> (Variant=w330:variant)  [unwired: 1 in]
                n124 = Unbundle By Name(w333) -> ()  [unwired: 1 out]
                n125 = Enqueue Element(queue=w331, element=w330, timeout in ms (-1)=100 ("超时毫秒(-1)")) -> ()  [unwired: 1 in, 3 out]
                n126 = property on="CFX_Message_In" class="Clust (严格)" props=["Value"]() -> ()  [unwired: 2 in, 3 out]
                n127 = property on="CFX_Message_In" class="Clust (严格)" props=["Value"](error in=w334) -> (error out=w335:errorcluster)  [unwired: 2 in, 1 out]
                n128 = call <vilib>:"Clear Errors.vi"("error in (no error)"=w335) -> ()  [unwired: 5 in, 2 out]
              }
              frame Enabled {
              }
            }
          }
        }
        n129 = Equal?(x=w294, y=w287) -> (x = y?=w289:bool)
        n130 = Select(t=w294, s=w289, f=w287) -> (s? t:f=w279:T1)
        n131 = Not(x=w282) -> (.not. x?=w264:bool)
        n132 = local read "MessageCFX_out"() -> (w293:string)
        n133 = Select(t=CFX-cmd."OpenConnection" ("CFX State"), s=w264, f=w279) -> (s? t:f=w278:T1)
      }
      frame "Shutdown" {
        n134 = Equal?(x=CfxTopic-cmd."EndpointShuttingDown" ("CFX cmd"), y=w339) -> (x = y?=w337:bool)
        n135 = case shown="True" w337 {
          tunnel: w346 -> [w349 w356]
          tunnel: [_ "关闭CFX通讯" ("格式字符串")] -> w345
          tunnel: [CFX-cmd."CFX" ("CFX State") w353] -> w344
          tunnel: w343 -> [w348 w372]
          tunnel: [w349 w355] -> w342
          tunnel: [w348 w354] -> w341
          tunnel: [_ TRUE] -> w340
          tunnel: [CfxTopic-cmd."EndpointShuttingDown" ("CFX cmd") _] -> w336
          frame False {
          }
          frame True {
            n136 = invoke on="调用节点" class="AmqpCFXEndpoint" method="Close"(reference=w356, error in=w372) -> (reference out=w370:refnum<k24>, error out=w371:errorcluster)  [unwired: 1 in, 1 out]
            n137 = invoke on="调用节点" class="AmqpCFXEndpoint" method="Dispose"(reference=w370, error in=w371) -> (reference out=w355:refnum<k24>, error out=w369:errorcluster)  [unwired: 1 in, 1 out]
            n138 = Close Reference(reference=w355, error in (no error)=w369) -> (error out=w364:errorcluster)
            n139 = call <vilib>:"Clear Errors.vi"("error in (no error)"=w364) -> ("error out"=w363:errorcluster)  [unwired: 5 in, 1 out]
            n140 = property on="TraceMessage_EVE" class="Ref (严格)"(error in=w363) -> (error out=w367:errorcluster, "Value"=w368:refnum<k27>)  [unwired: 1 in, 1 out]
            n141 = Unregister For Events(event registration refnum=w368, error in=w367) -> (error out=w362:errorcluster)
            n142 = property on="objAMQP_MSG" class="Ref (严格)"(error in=w362) -> (error out=w361:errorcluster, "Value"=w360:refnum<k27>)  [unwired: 1 in, 1 out]
            n143 = Unregister For Events(event registration refnum=w360, error in=w361) -> (error out=w359:errorcluster)
            n144 = property on="objAMQP_Request" class="Ref (严格)"(error in=w359) -> (error out=w358:errorcluster, "Value"=w357:refnum<k27>)  [unwired: 1 in, 1 out]
            n145 = property on="ok?" class="Bool (严格)"() -> ("Value"=w352:bool)  [unwired: 2 in, 2 out]
            n146 = Unregister For Events(event registration refnum=w357, error in=w358) -> (error out=w366:errorcluster)
            n147 = call <vilib>:"Clear Errors.vi"("error in (no error)"=w366) -> ("error out"=w354:errorcluster)  [unwired: 5 in, 1 out]
            n148 = Select(t=CFX-cmd."Shutdown" ("CFX State"), s=w352, f=CFX-cmd."Initialize") -> (s? t:f=w353:T1)
          }
        }
      }
      frame "WorkComplete" {
        w398 = 0 items=["Completed", "Failed", ""] ("Result")
        n149 = constructor class="WorkStarted"(error in=w376) -> (reference out=w399:refnum<k24>, error out=w396:errorcluster)  [unwired: 2 in, 1 out]
        n150 = property class="WorkStarted"(reference=w399, error in=w396) -> (error out=w395:errorcluster, "TransactionID"=w397:refnum<k24>)  [unwired: 1 out]
        n151 = constructor class="WorkCompleted"(error in=w395) -> (reference out=w394:refnum<k24>, error out=w393:errorcluster)  [unwired: 2 in, 1 out]
        n152 = property class="WorkCompleted"(reference=w394, error in=w393, "Result"=w398, "TransactionID"=w397) -> (reference out=w384:refnum<k24>, error out=w392:errorcluster)
        n153 = constructor class="CFXEnvelope"() -> (reference out=w401:refnum<k24>, error out=w400:errorcluster)  [unwired: 3 in, 1 out]
        n154 = property class="CFXEnvelope"(reference=w401, error in=w400, "MessageBody"=w384) -> (reference out=w387:refnum<k24>, error out=w388:errorcluster, "MessageName"=w382:string)
        n155 = invoke class="AmqpCFXEndpoint" method="Publish"(reference=w390, error in=w392, "env"=w387) -> (reference out=w389:refnum<k24>, error out=w391:errorcluster)  [unwired: 1 in, 2 out]
        n156 = invoke on="调用节点" class="CFXJsonSerializer" method="SerializeObjectWithTypes"("o"=w384, "formatted"=TRUE) -> (reference out=w383:refnum<k24>, error out=w385:errorcluster, "SerializeObjectWithTypes"=w381:string)  [unwired: 3 in, 2 out]
        n157 = Close Reference(reference=w383, error in (no error)=w385) -> (error out=w379:errorcluster)
        n158 = Merge Errors(w391, w388) -> (w386:errorcluster)
        n159 = Format Into String(format string="\n-------- Message Content --------\n%s" ("格式字符串"), initial string=w382, error in=w379, w381) -> (resulting string=w378:string)  [unwired: 1 out]
      }
      frame "StationStateChanged" {
        n160 = constructor class="StationStateChanged"(error in=w403) -> (reference out=w423:refnum<k24>, error out=w422:errorcluster)  [unwired: 2 in, 1 out]
        n161 = local read "rngNewState"() -> (w417:i32)
        n162 = property class="StationStateChanged"(reference=w423, error in=w422, "NewState"=w417) -> (reference out=w409:refnum<k24>, error out=w419:errorcluster)
        n163 = constructor class="CFXEnvelope"() -> (reference out=w420:refnum<k24>, error out=w421:errorcluster)  [unwired: 3 in, 1 out]
        n164 = property class="CFXEnvelope"(reference=w420, error in=w421, "MessageBody"=w409) -> (reference out=w412:refnum<k24>, error out=w414:errorcluster, "MessageName"=w407:string)
        n165 = invoke class="AmqpCFXEndpoint" method="Publish"(reference=w418, error in=w419, "env"=w412) -> (reference out=w416:refnum<k24>, error out=w415:errorcluster)  [unwired: 1 in, 2 out]
        n166 = invoke on="调用节点" class="CFXJsonSerializer" method="SerializeObjectWithTypes"("o"=w409, "formatted"=TRUE) -> (reference out=w411:refnum<k24>, error out=w410:errorcluster, "SerializeObjectWithTypes"=w405:string)  [unwired: 3 in, 2 out]
        n167 = Close Reference(reference=w411, error in (no error)=w410) -> (error out=w406:errorcluster)
        n168 = Merge Errors(w415, w414) -> (w413:errorcluster)
        n169 = Format Into String(format string="\n-------- Message Content --------%s" ("格式字符串"), initial string=w407, error in=w406, w405) -> ()  [unwired: 2 out]
      }
      frame "MaterialsApplied" {
        n170 = constructor class="MaterialsApplied"(error in=w425) -> (reference out=w448:refnum<k24>, error out=w450:errorcluster)  [unwired: 2 in, 1 out]
        n171 = constructor class="InstalledMaterial"() -> (reference out=w446:refnum<k24>, error out=w447:errorcluster)  [unwired: 3 in, 1 out]
        n172 = invoke class="Guid" method="NewGuid"(error in=w450) -> (error out=w451:errorcluster, "NewGuid"=w449:refnum<k24>)  [unwired: 2 in, 1 out]
        n173 = property class="MaterialsApplied"(reference=w448, error in=w451, "TransactionId"=w449) -> (reference out=w457:refnum<k24>, error out=w438:errorcluster, "AppliedMaterials"=w452:refnum<k24>)
        n174 = property class="InstalledMaterial"(reference=w446, error in=w447, "QuantityInstalled"=1.0, "QuantityNonInstalled"=2.0) -> (reference out=w453:refnum<k24>, error out=w435:errorcluster)
        n175 = Merge Errors(w438, w435) -> (w436:errorcluster)
        n176 = invoke class="List`1[[CFX.Structures.Installe" method="Add"(reference=w452, error in=w436, "item"=w453) -> (reference out=w454:refnum<k24>, error out=w437:errorcluster)  [unwired: 1 in, 2 out]
        n177 = property class="MaterialsApplied"(reference=w457, error in=w437, "AppliedMaterials"=w454) -> (reference out=w431:refnum<k24>, error out=w439:errorcluster)
        n178 = constructor class="CFXEnvelope"(error in=w439) -> (reference out=w455:refnum<k24>, error out=w456:errorcluster)  [unwired: 2 in, 1 out]
        n179 = property class="CFXEnvelope"(reference=w455, error in=w456, "MessageBody"=w431) -> (reference out=w434:refnum<k24>, error out=w440:errorcluster, "MessageName"=w429:string)
        n180 = invoke class="AmqpCFXEndpoint" method="Publish"(reference=w443, error in=w440, "env"=w434) -> (reference out=w442:refnum<k24>, error out=w441:errorcluster)  [unwired: 1 in, 2 out]
        n181 = invoke on="调用节点" class="CFXJsonSerializer" method="SerializeObjectWithTypes"("o"=w431, "formatted"=TRUE) -> (reference out=w432:refnum<k24>, error out=w433:errorcluster, "SerializeObjectWithTypes"=w428:string)  [unwired: 3 in, 2 out]
        n182 = Close Reference(reference=w432, error in (no error)=w433) -> ()  [unwired: 1 out]
        n183 = Format Into String(format string="\n-------- Message Content --------\n%s" ("格式字符串"), initial string=w429, w428) -> (resulting string=w427:string)  [unwired: 1 in, 1 out]
      }
      frame "CFX" {
        w462 = CfxTopic-cmd."EndpointShuttingDown" ("CFX cmd")
        n184 = First Call?() -> (First Call?: T/F=w472:bool)
        n185 = Not Equal?(x=w467, y=CfxTopic-cmd."AreYouThereRequest" ("CFX cmd")) -> (x != y?=w473:bool)
        n186 = Equal?(x=w462, y=w467) -> (x = y?=w466:bool)
        n187 = Or(x=w473, y=w472) -> (x .or. y?=w474:bool)
        n188 = case shown="False" w474 {
          tunnel: w467 -> [_ w495]
          tunnel: ["CFX cmd" w495] -> w475
          frame False {
          }
          frame True {
          }
        }
        n189 = property on="return" class="Clust (严格)"() -> ("Value"=w471:T6)  [unwired: 2 in, 2 out]
        n190 = Unbundle By Name(w471) -> ("CFXHandle"=w470:string, "RequestNetworkUri"=w469:string, "RequestTargetAddress"=w468:string)
        n191 = property on="EndpointInformation" class="Str"(error in=w484) -> (error out=w489:errorcluster, "Value"=w492:string)  [unwired: 1 in, 1 out]
        n192 = call "_lcod_CFX.vi"("RequestTargetAddress"=w468, "RequestNetworkUri"=w469, "cmd"=w475, "Error In"=w489, "in_str"=w492, "CFXHandle"=w470, "CfxData"="CfxData") -> ("Error Out"=w461:errorcluster, "new reference"=w480:refnum<k24>)  [unwired: 2 in, 1 out]
        n193 = Get Date/Time In Seconds() -> (seconds since 1Jan1904=w485:timestamp)
        n194 = property class="CFXEnvelope"(reference=w480, error in=w461, "Source"=w460, "Target"=w459, "TimeStamp"=w485) -> (reference out=w479:refnum<k24>, error out=w486:errorcluster, "MessageName"=w478:string)
        n195 = invoke class="AmqpCFXEndpoint" method="Publish"(reference=w483, error in=w486, "env"=w479) -> (reference out=w482:refnum<k24>, error out=w493:errorcluster)  [unwired: 1 in, 2 out]
        n196 = invoke on="调用节点" class="CFXJsonSerializer" method="SerializeObjectWithTypes"("o"=w479, "formatted"=TRUE) -> (reference out=w490:refnum<k24>, error out=w491:errorcluster, "SerializeObjectWithTypes"=w477:string)  [unwired: 3 in, 2 out]
        n197 = Close Reference(reference=w490, error in (no error)=w491) -> ()  [unwired: 1 out]
        n198 = Format Into String(format string="Direction: Send | %s\n-------- Message Content -------\n%s" ("格式字符串"), w478, w477) -> (resulting string=w487:string)  [unwired: 2 in, 1 out]
        n199 = Select(t=CFX-cmd."Shutdown" ("CFX State"), s=w466, f=CFX-cmd."Idle" ("CFX State")) -> (s? t:f=w463:T1)
      }
      frame "Hermes" {
        n200 = disable-structure shown="禁用" {
          disable-tunnel: w501 -> [w504 w506]
          disable-tunnel: [w503 w506] -> w500
          disable-tunnel: [w502 w505] -> w499
          disable-tunnel: [_ ""] -> w498
          disable-tunnel: w496 -> [_ w505]
          frame Disabled {
            n201 = invoke class="AmqpCFXEndpoint" method="Publish"(reference=w504) -> (reference out=w503:refnum<k24>, error out=w502:errorcluster)  [unwired: 3 in, 2 out]
          }
          frame Enabled {
          }
        }
      }
    }
    "MessageCFX_out" <- w68
    "cmd State" <- w47
    n202 = Call Chain() -> (call chain=w52:string[])
    n203 = Array Size(array=w52) -> (size(s)=w51:i32)
    n204 = Empty String/Path?(string/path=w67) -> (empty?=w66:bool)
    n205 = Equal?(x=w47, y=w35) -> (x = y?=w44:bool)
    n206 = Greater?(x=w51, y=1) -> (0:w45:bool)
    n207 = case shown="False" w66 {
      tunnel: w69 -> [w90 w92]
      tunnel: [w89 w91] -> w64
      tunnel: w67 -> [w84 _]
      tunnel: w39 -> [w82 _]
      frame False {
        n208 = call "Cfx_log.vi"("login"=w84, "error in"=w90, "log_path"=w82) -> ("Log_out"=w83:string, "error out"=w89:errorcluster)  [unwired: 15 in]
        n209 = Format Into String(format string="CFX . 执行信息】\n消息：%s", w83) -> (resulting string=w87:string, error out=w88:errorcluster)  [unwired: 2 in]
        n210 = call "lcod run log.vi"("cmd"=_myType_runlog_cmd."push (1: logical)", "Error In"=w88, "str in"=w87) -> ()  [unwired: 6 in, 3 out]
        "log" <- w84
      }
      frame True {
        n211 = call <vilib>:"Simple Error Handler.vi"("error in (no error)"=w92) -> ("error out"=w91:errorcluster)  [unwired: 4 in, 4 out]
      }
    }
    "error out" <- w64
    n212 = Compound Arithmetic op=AND ("复合运算")(w44, w45) -> (w46:bool)
    n213 = case shown="True" w46 {
      tunnel: w49 -> [w77 w79]
      tunnel: [w77 w80] -> w48
      tunnel: [_ w78] -> w37
      frame False {
        n214 = Wait (ms)(milliseconds to wait=u32 10 ("等待时间（毫秒）")) -> ()  [unwired: 1 out]
      }
      frame True {
        n215 = call "lcod exit.vi"() -> ("bExit out"=w78:bool)  [unwired: 11 in]
        n216 = Select(t=w79, s=w78, f=TRUE) -> (s? t:f=w80:bool)
      }
    }
    n217 = Or(x=w48, y=w31) -> (x .or. y?=w32:bool)
  }
  n218 = case shown="False" w3 {
    tunnel: w6 -> [w512 _]
    tunnel: w5 -> [w511 _]
    tunnel: w4 -> [w510 _]
    tunnel: w2 -> [w509 _]
    tunnel: w1 -> [w508 _]
    frame False {
      n219 = while {
        shift-right: [w541] -> _
        shift-left: _ -> [w540]
        shift-right: [w539] -> _
        shift-left: _ -> [w528]
        shift-right: [w538] -> _
        shift-left: _ -> [w537]
        tunnel: w512 -> [w523]
        tunnel: w511 -> [w519]
        shift-right: [w536] -> _
        shift-left: _ -> [w535]
        shift-right: [w533] -> _
        shift-left: _ -> [w534]
        tunnel: w510 -> [w532]
        shift-right: [w516] -> _
        shift-left: _ -> [w515]
        tunnel: w509 -> [w514]
        tunnel: w508 -> [w513]
        stop <- w517 stop-if-true
        # "CFX监听点对点消息&请求CFX.Handle消息"
        n220 = First Call?() -> (First Call?: T/F=w529:bool)
        n221 = case shown="True" w529 {
          tunnel: [_ w551] -> w520
          frame False {
          }
          frame True {
            n222 = call "时间延迟"() -> ("error out"=w551:errorcluster)  [unwired: 11 in]
          }
        }
        n223 = First Call?() -> (First Call?: T/F=w543:bool)
        n224 = Format Into String(format string="CFX_%s" ("log_path"), w519) -> (resulting string=w521:string)  [unwired: 2 in, 1 out]
        n225 = Select(t=CFX-cmd."Initialize" ("CFX State"), s=w543, f=w534) -> (s? t:f=w542:T1)
        n226 = case shown="\"Idle\"" w542 {
          tunnel: [w566 w581 w593 w609 w627 w691] -> w541
          tunnel: w540 -> [w565 w581 w601 w620 w642 w697]
          tunnel: [w563 w575 w594 w617 w628 w692] -> w539
          tunnel: w528 -> [_ w578 w590 w619 w641 _]
          tunnel: [_ w580 w592 w616 w640 _] -> w538
          tunnel: w537 -> [_ w579 w592 w616 w640 w695]
          tunnel: w523 -> [_ _ w600 _ _ _]
          tunnel: ["初始化CFX监听节点" ("格式字符串") "CFX注册回调事件" ("格式字符串") w591 "打开监听节点连接" ("格式字符串") w621 "关闭CFX监听实例" ("格式字符串")] -> w530
          tunnel: w519 -> [_ _ _ w618 w625 _]
          tunnel: [w560 w572 w588 w615 w633 w687] -> w536
          tunnel: w535 -> [w560 w572 _ w615 w633 w687]
          tunnel: [CFX-cmd."Event" ("CFX State") CFX-cmd."Connection test" ("CFX State") CFX-cmd."OpenConnection" ("CFX State") CFX-cmd."Idle" ("CFX State") w634 CFX-cmd."Shutdown" ("f")] -> w533
          tunnel: w532 -> [_ _ _ w612 w624 _]
          tunnel: [_ _ _ _ _ TRUE] -> w518
          tunnel: w520 -> [_ _ _ _ _ _]
          tunnel: w514 -> [_ _ _ _ w626 _]
          tunnel: w513 -> [_ _ _ _ w622 _]
          frame "Initialize", Default {
            n227 = invoke class="AmqpCFXEndpoint" method="Close"(reference=w565) -> (reference out=w570:refnum<k24>, error out=w568:errorcluster)  [unwired: 2 in, 1 out]
            n228 = invoke on="调用节点" class="AmqpCFXEndpoint" method="Dispose"(reference=w570, error in=w568) -> (reference out=w567:refnum<k24>, error out=w569:errorcluster)  [unwired: 1 in, 1 out]
            n229 = Close Reference(reference=w567, error in (no error)=w569) -> (error out=w571:errorcluster)
            n230 = call <vilib>:"Clear Errors.vi"("error in (no error)"=w571) -> ("error out"=w564:errorcluster)  [unwired: 5 in, 1 out]
            n231 = constructor class="AmqpCFXEndpoint"(error in=w564) -> (reference out=w566:refnum<k24>, error out=w563:errorcluster)  [unwired: 2 in, 1 out]
          }
          frame "Event" {
            n232 = Unregister For Events(event registration refnum=w579, error in=w578) -> (error out=w577:errorcluster)
            n233 = call <vilib>:"Clear Errors.vi"("error in (no error)"=w577) -> ("error out"=w576:errorcluster)  [unwired: 5 in, 1 out]
            n234 = vi-ref "OnRequestReceived.vi"() -> ("vi reference"=w585:refnum<vi>)
            n235 = vi-ref "OnConnectionEvent.vi"() -> ("vi reference"=w583:refnum<vi>)
            n236 = control-ref of="return"() -> (w584:refnum<vi>)
            n237 = control-ref of="Connection"() -> (w582:refnum<vi>)
            n238 = node(w576, w581, w585, w584, w581, w583, w582) -> (w580:refnum<k27>, w575:errorcluster)  [unwired: 1 in]
          }
          frame "Connection test" {
            n239 = call <vilib>:"Clear Errors.vi"("error in (no error)"=w590) -> ("error out"=w586:errorcluster)  [unwired: 5 in, 1 out]
            n240 = constructor class="Uri"(error in=w586, "uriString"=w600) -> (reference out=w588:refnum<k24>, error out=w589:errorcluster)  [unwired: 2 in, 2 out]
            n241 = invoke on="调用节点" class="AmqpCFXEndpoint" method="TestChannel"(reference=w601, error in=w589, "channelUri"=w588) -> (reference out=w593:refnum<k24>, error out=w594:errorcluster, "error"=w599:refnum<k24>)  [unwired: 3 in, 3 out]
            n242 = invoke class="Exception" method="ToString"(reference=w599) -> (reference out=w598:refnum<k24>, error out=w595:errorcluster, "ToString"=w597:string)  [unwired: 2 in]
            n243 = case shown="无错误" w595 {
              tunnel: "objAMQP_Request" ("格式字符串") -> [w605 w608]
              tunnel: [w604 w608] -> w591
              tunnel: w597 -> [w602 _]
              tunnel: w598 -> [_ w607]
              frame No Error {
                n244 = Format Into String(format string="监听监控：%s" ("格式字符串"), initial string=w605, w602) -> (resulting string=w604:string)  [unwired: 1 in, 1 out]
              }
              frame Error {
                n245 = Close Reference(reference=w607) -> (error out=w606:errorcluster)  [unwired: 1 in]
                n246 = call <vilib>:"Clear Errors.vi"("error in (no error)"=w606) -> ()  [unwired: 5 in, 2 out]
              }
            }
          }
          frame "OpenConnection" {
            n247 = invoke class="AmqpCFXEndpoint" method="Open"(reference=w620, error in=w619, "cfxHandle"=w618, "requestUri"=w615) -> (reference out=w610:refnum<k24>, error out=w617:errorcluster)  [unwired: 2 in, 4 out]
            n248 = invoke class="TimeSpan" method="FromSeconds"("value"=w612) -> ("FromSeconds"=w613:refnum<k24>)  [unwired: 3 in, 3 out]
            n249 = property on="属性节点" class="AmqpCFXEndpoint"(reference=w610, "RequestTimeout"=w613) -> (reference out=w609:refnum<k24>)  [unwired: 1 in, 1 out]
          }
          frame "Idle" {
            w636 = CFX-cmd."Shutdown" ("y")
            n250 = property on="属性节点" class="AmqpCFXEndpoint"(reference=w642, error in=w641) -> (reference out=w630:refnum<k24>, error out=w629:errorcluster, "IsOpen"=w632:bool)
            "IsOpen" <- w632
            n251 = case shown="False" "request?" {
              tunnel: w630 -> [w644 w686]
              tunnel: w629 -> [w643 w647]
              tunnel: [w643 w645] -> w628
              tunnel: [w644 w685] -> w627
              tunnel: w626 -> [_ w684]
              tunnel: w625 -> [_ w654]
              tunnel: w624 -> [_ w676]
              tunnel: w622 -> [_ w653]
              tunnel: [_ w650] -> w621
              frame False {
              }
              frame True {
                n252 = property on="CFX cmd" class="Enum (严格)"(error in=w647) -> (error out=w648:errorcluster, "Value"=w667:T7)  [unwired: 1 in, 1 out]
                n253 = property on="return" class="Clust (严格)"() -> ("Value"=w668:T6)  [unwired: 2 in, 2 out]
                n254 = property on="EndpointInformation" class="Str"() -> ("Value"=w672:string)  [unwired: 2 in, 2 out]
                n255 = Unbundle By Name(w668) -> ("CFXHandle"=w671:string, "RequestNetworkUri"=w670:string, "RequestTargetAddress"=w669:string)
                n256 = property on="request?" class="Bool (严格)"(error in=w648, "Value"=FALSE ("request?")) -> (error out=w649:errorcluster)  [unwired: 1 in, 1 out]
                n257 = local read "CfxData"() -> (w666:T2)
                n258 = call "_lcod_CFX.vi"("RequestTargetAddress"=w669, "RequestNetworkUri"=w670, "cmd"=w667, "in_str"=w672, "CFXHandle"=w671, "CfxData"=w666) -> ("new reference"=w665:refnum<k24>)  [unwired: 3 in, 2 out]
                n259 = Get Date/Time In Seconds() -> (seconds since 1Jan1904=w652:timestamp)
                n260 = property class="CFXEnvelope"(reference=w665, "Source"=w654, "Target"=w653, "TimeStamp"=w652) -> (reference out=w664:refnum<k24>, error out=w651:errorcluster, "MessageName"=w660:string)  [unwired: 1 in]
                n261 = invoke on="调用节点" class="CFXJsonSerializer" method="SerializeObjectWithTypes"(error in=w651, "o"=w664, "formatted"=TRUE) -> (reference out=w659:refnum<k24>, error out=w658:errorcluster, "SerializeObjectWithTypes"=w661:string)  [unwired: 2 in, 2 out]
                n262 = invoke on="调用节点" class="AmqpCFXEndpoint" method="ExecuteRequestAsync"(reference=w686, error in=w649, "targetUri"=w684, "request"=w664) -> (reference out=w685:refnum<k24>, error out=w646:errorcluster, "ExecuteRequestAsync"=w677:refnum<k24>)  [unwired: 1 in, 2 out]
                n263 = Close Reference(reference=w659, error in (no error)=w658) -> (error out=w657:errorcluster)
                n264 = vi-ref "_lcod_CFX_ExecuteReguestAsync.vi"() -> (w682:refnum<vi>)
                n265 = Format Into String(format string="Direction: EQ_request_Send | %s\n-------- Message Content -------\n%s" ("格式字符串"), error in=w657, w660, w661) -> (resulting string=w650:string, error out=w655:errorcluster)  [unwired: 1 in]
                n266 = property class="VI接口类型0"(reference=w682) -> (error out=w680:errorcluster, "Path"=w683:path)  [unwired: 1 in, 1 out]
                n267 = Open VI Reference(type specifier VI Refnum (for type only)=w682, vi path=w683, options=128 ("选项"), error in (no error)=w680) -> (vi reference=w681:refnum<vi>, error out=w679:errorcluster)  [unwired: 2 in]
                n268 = control-ref of="CFX_Message_In"() -> (w675:refnum<vi>)
                n269 = call-by-ref "开始异步调用"(reference=w681, error in=w679, "CFX_Message"=w675, "timeout"=w676, "Handle"=w654, "ExecuteReouestAsync"=w677) -> (error out=w674:errorcluster)  [unwired: 7 in, 2 out]
                n270 = Merge Errors(w646, w674, w655) -> (w656:errorcluster)
                n271 = call <vilib>:"Clear Errors.vi"("error in (no error)"=w656) -> ("error out"=w645:errorcluster)  [unwired: 5 in, 1 out]
              }
            }
            n272 = property on="cmd State" class="Enum (严格)"() -> ("Value"=w631:T1)  [unwired: 2 in, 2 out]
            n273 = Equal?(x=w636, y=w631) -> (x = y?=w637:bool)
            n274 = Select(t=CFX-cmd."Idle" ("f"), s=w632, f=CFX-cmd."Connection test") -> (s? t:f=w635:T1)
            n275 = Select(t=w636, s=w637, f=w635) -> (s? t:f=w634:T1)
          }
          frame "Shutdown" {
            n276 = invoke on="调用节点" class="AmqpCFXEndpoint" method="Close"(reference=w697) -> (reference out=w699:refnum<k24>, error out=w700:errorcluster)  [unwired: 2 in, 1 out]
            n277 = invoke on="调用节点" class="AmqpCFXEndpoint" method="Dispose"(reference=w699, error in=w700) -> (reference out=w691:refnum<k24>, error out=w698:errorcluster)  [unwired: 1 in, 1 out]
            n278 = Close Reference(reference=w691, error in (no error)=w698) -> (error out=w696:errorcluster)
            n279 = call <vilib>:"Clear Errors.vi"("error in (no error)"=w696) -> ("error out"=w694:errorcluster)  [unwired: 5 in, 1 out]
            n280 = Unregister For Events(event registration refnum=w695, error in=w694) -> (error out=w693:errorcluster)
            n281 = call <vilib>:"Clear Errors.vi"("error in (no error)"=w693) -> ("error out"=w692:errorcluster)  [unwired: 5 in, 1 out]
          }
        }
        n282 = Empty String/Path?(string/path=w530) -> (empty?=w531:bool)
        n283 = Call Chain() -> (call chain=w527:string[])
        n284 = case shown="False" w531 {
          tunnel: w530 -> [w555 _]
          tunnel: w521 -> [w556 _]
          frame False {
            n285 = call "Cfx_log.vi"("login"=w555, "log_path"=w556) -> ("Log_out"=w553:string, "error out"=w554:errorcluster)  [unwired: 16 in]
            n286 = Format Into String(format string="CFX . 执行信息】\n消息：%s", w553) -> (resulting string=w557:string)  [unwired: 2 in, 1 out]
            n287 = call "lcod run log.vi"("cmd"=_myType_runlog_cmd."push (1: logical)", "Error In"=w554, "str in"=w557) -> ("Error Out"=w552:errorcluster)  [unwired: 6 in, 2 out]
            n288 = call <vilib>:"Clear Errors.vi"("error in (no error)"=w552) -> ()  [unwired: 5 in, 2 out]
          }
          frame True {
          }
        }
        n289 = Array Size(array=w527) -> (size(s)=w526:i32)
        n290 = Greater?(x=w526, y=1) -> (0:w522:bool)
        n291 = case shown="False" w522 {
          tunnel: w518 -> [w545 _]
          tunnel: [w545 w549] -> w517
          tunnel: [_ w548] -> w516
          tunnel: w515 -> [_ w547]
          frame False {
            n292 = Wait (ms)(milliseconds to wait=u32 100 ("等待时间（毫秒）")) -> ()  [unwired: 1 out]
          }
          frame True {
            n293 = call "lcod exit.vi"() -> ("bExit out"=w548:bool)  [unwired: 11 in]
            n294 = Select(t=w547, s=w548, f=TRUE) -> (s? t:f=w549:bool)
          }
        }
      }
    }
    frame True {
    }
  }
  n295 = Bundle By Name(cluster=w13, "CFX_Handle"=w5) -> (→"CFX_Message_In":T4)
  n296 = disable-structure shown="禁用" {
    frame Disabled {
      (unwired) "/queue/Cleaner" ("RequestTargetAddress")
      (unwired) 0 items=["ConnectionEstablished", "ConnectionFailed", "ConnectionInterrupted", "ConnectionClosed"] ("ConnectionEstablished")
      n297 = invoke on="调用节点" class="CFXJsonSerializer" method="DeserializeObject"() -> ()  [unwired: 5 in, 5 out]
      n298 = constructor class="EndpointConnected"() -> (reference out=w706:refnum<k24>, error out=w707:errorcluster)  [unwired: 3 in, 1 out]
      n299 = invoke class="Dns" method="GetHostName"() -> ()  [unwired: 3 in, 3 out]
      n300 = invoke class="Dns" method="GetHostName"() -> (error out=w711:errorcluster, "GetHostName"=w708:string)  [unwired: 3 in, 1 out]
      n301 = Concatenate Strings("amqp://") -> ()  [unwired: 1 in, 1 out]
      n302 = invoke on="调用节点" class="EndpointConnected" method="GetHashCode"(reference=w706, error in=w707) -> ()  [unwired: 1 in, 3 out]
      n303 = invoke on="调用节点" class="AmqpCFXEndpoint" method="ExecuteRequestAsync"() -> ()  [unwired: 5 in, 5 out]
      n304 = constructor class="UriFormat"(error in=w711) -> (reference out=w713:refnum<k24>, error out=w712:errorcluster)  [unwired: 2 in, 1 out]
      n305 = Concatenate Strings("amqp://localhost:5672/#/" ("format"), w708) -> (w709:string)
      n306 = property class="EndpointConnected" props=["RequestNetworkUri"]() -> ()  [unwired: 3 in, 2 out]
      n307 = invoke class="UriFormat" method="ToString"(reference=w713, error in=w712, "format"=w709) -> ()  [unwired: 1 in, 4 out]
      n308 = property class="CFXJsonSerializer" props=["JsonSettings"]() -> ()  [unwired: 3 in, 2 out]
      n309 = constructor class="AppLogSettings"() -> ()  [unwired: 3 in, 3 out]
      n310 = call "_lcod_CFX_ExecuteReguestAsync.vi"() -> ("CFX_Message_out"=w701:T4)  [unwired: 11 in]
      n311 = invoke on="调用节点" class="CFXJsonSerializer" method="SerializeObjectWithTypes"() -> (reference out=w704:refnum<k24>, error out=w705:errorcluster)  [unwired: 5 in, 3 out]
      n312 = property on="CFX_Message_In" class="Clust (严格)"("Value"=w701) -> ()  [unwired: 2 in, 2 out]
      n313 = call "lcod log for app error.vi"() -> ()  [unwired: 10 in, 2 out]
      n314 = Format Into String() -> ()  [unwired: 4 in, 2 out]
      n315 = Close Reference(reference=w704, error in (no error)=w705) -> ()  [unwired: 1 out]
      n316 = Format Into String(format string="-------- Message Content --------\n%s" ("格式字符串")) -> ()  [unwired: 3 in, 2 out]
    }
    frame Enabled {
    }
  }
  n317 = Merge Errors("Error In", w7) -> (→"Error Out":errorcluster)
